vi "Locate Time.vi"(10 "Date":timestamp, 11 "Date Array":timestamp[](array[timestamp])) -> (3 "Index":i32)   [LabVIEW 2020, in "Data Viewer.lvlib" / "Data Viewer.lvclass"]
uses:
  Data Viewer.lvclass
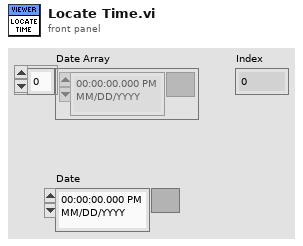
[diagram p1: front panel]
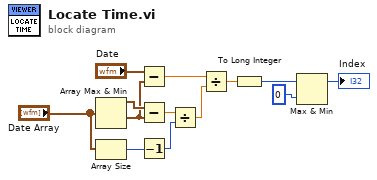
[diagram p0: block diagram]
diagram:
  n1 = Array Max & Min(array="Date Array") -> (max value=w13:timestamp, min value=w7:timestamp)  [unwired: 2 out]
  n2 = Array Size(array="Date Array") -> (size(s)=w10:i32)
  n3 = Subtract(x="Date", y=w7) -> (x-y=w5:dbl)
  n4 = Subtract(x=w13, y=w7) -> (x-y=w12:dbl)
  n5 = Decrement(x=w10) -> (x-1=w9:i32)
  n6 = Divide(x=w12, y=w9) -> (x/y=w6:dbl)
  n7 = Divide(x=w5, y=w6) -> (x/y=w4:dbl)
  n8 = To Long Integer(number=w4) -> (32bit integer=w3:i32)
  n9 = Max & Min(x=w3, y=0) -> (max(x,y)=→"Index":i32)  [unwired: 1 out]
